vi "G-Uart-Push_data.vi"(8 "error in (no error)":errorcluster caption="错误输入（无错误）", 9 "写入缓冲区":string, 10 "Uart":T1, 11 "G-Uart-Class 输入":refnum<class "G-Uart-Class.lvclass">) -> (0 "error out":errorcluster caption="错误输出", 3 "G-Uart-Class 输出":refnum<class "G-Uart-Class.lvclass">)   [LabVIEW 2025, in "G-Uart-Class.lvclass"]
uses:
  G-Uart-Class.lvclass
  Register-Uart.ctl
  G-Uart-Class.lvclass/G-Uart-Class.ctl
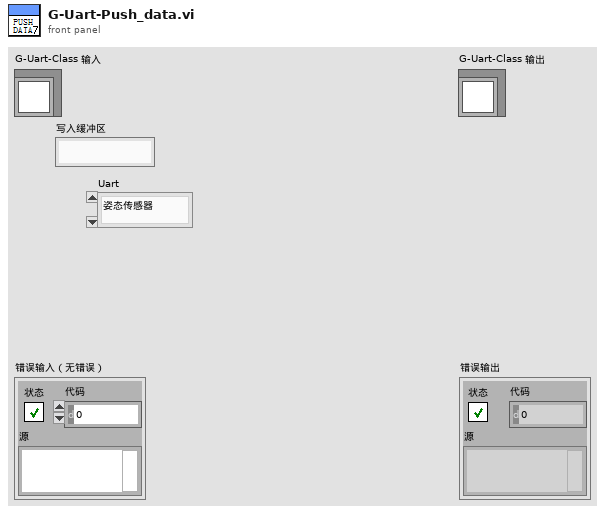
[diagram p1: front panel]
types:
  T1 = typedef "G-Uart-Class.lvclass/Register-Uart.ctl" = enum16{"姿态传感器", "图像跟踪", "观瞄仪器", "电源"}
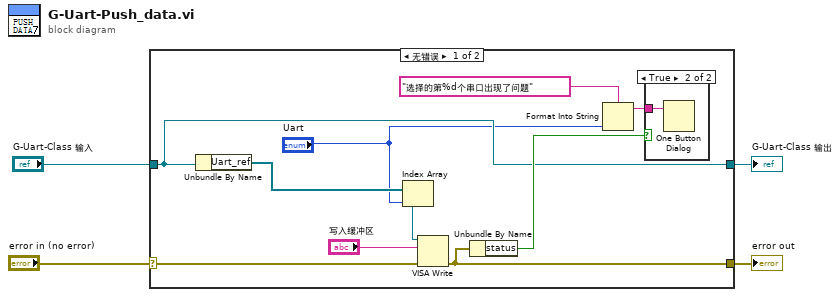
[diagram p0: block diagram]
diagram:
  n1 = case shown="无错误" "error in (no error)" {
    selector: "error in (no error)" -> [w12 w17]
    tunnel: [w10 w17] -> w3
    tunnel: [w7 w16] -> w1
    tunnel: "G-Uart-Class 输入" -> [w7 w16]
    frame No Error {
      n2 = Unbundle By Name(w7) -> ("Uart_ref"=w6:refnum<visa-resource-name>[])
      n3 = Index Array(array=w6, index="Uart") -> (element=w14:refnum<visa-resource-name>)
      n4 = VISA Write(VISA resource name=w14, write buffer="写入缓冲区", error in (no error)=w12) -> (error out=w10:errorcluster)  [unwired: 2 out]
      n5 = Unbundle By Name(w10) -> ("status"=w11:bool)
      n6 = Format Into String(format string="选择的第%d个串口出现了问题" ("格式字符串"), "Uart") -> (resulting string=w8:string)  [unwired: 2 in, 1 out]
      n7 = case shown="True" w11 {
        tunnel: w8 -> [_ w15]
        frame False {
        }
        frame True {
          n8 = One Button Dialog(message=w15) -> ()  [unwired: 1 in, 1 out]
        }
      }
    }
    frame Error {
    }
  }
  "error out" <- w3
  "G-Uart-Class 输出" <- w1
